vi "Create.vi"(6 "Label Names":string[](array[string]), 7 "Registry Name":string, 8 "error in (no error)":errorcluster) -> (0 "error out":errorcluster, 3 "Process Collector out":refnum<class "Process Collector.lvclass">)   [LabVIEW 2020, in "Collector.lvlib" / "Process Collector.lvclass"]
doc: "Creates a collector for the hosting process. This collector contains CPU and memory information about the process running this code."
uses:
  Process Collector.lvclass
  Process Collector.lvclass/Process Collector.ctl
  metrics/gauge/Gauge.lvclass
  C:/Github-locals/PromVIEW/src/metrics/metric/Metric.lvclass
  <vilib>/regexp/Match Regular Expression.xnode
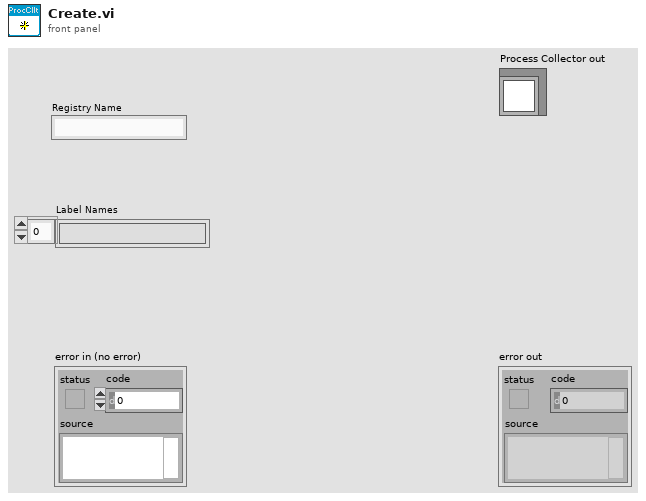
[diagram p1: front panel]
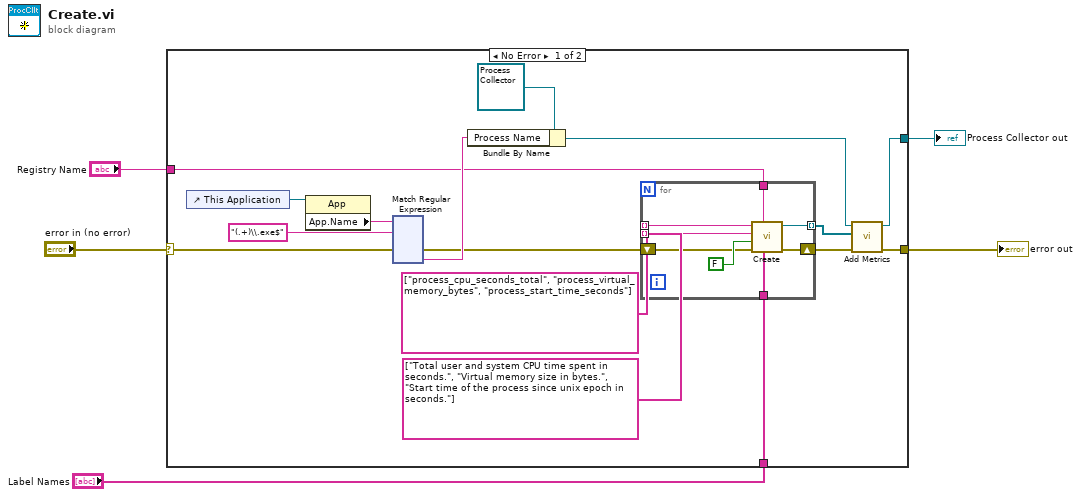
[diagram p0: block diagram]
diagram:
  n1 = case shown="No Error" "error in (no error)" {
    selector: "error in (no error)" -> [w17 w146]
    tunnel: [w8 w146] -> w2
    tunnel: [w9 _] -> w3
    tunnel: "Registry Name" -> [w13 _]
    tunnel: "Label Names" -> [w6 _]
    frame No Error {
      n2 = control-ref of="This Application"() -> (w21:refnum<vi>)
      n3 = property class="App"(reference=w21) -> ("App.Name"=w20:string)  [unwired: 1 in, 2 out]
      n4 = xnode "Match Regular Expression"("input string"=w20, "regular expression"="(.+)\\.exe$", "error in"=w17) -> ("error out"=w12:errorcluster, "submatch 1"=w18:string)  [unwired: 3 in, 4 out]
      n5 = Bundle By Name(cluster=refnum<class "Process Collector.lvclass"> refnum ("Process Collector in"), "Process Name"=w18) -> (w10:refnum<class "Process Collector.lvclass">)
      n6 = for {
        tunnel: string[] ["process_cpu_seconds_total", "process_virtual_memory_bytes", "process_start_time_seconds"] ("Metric Name") -> [w29] mode=indexing
        tunnel: string[] ["Total user and system CPU time spent in seconds.", "Virtual memory size in bytes.", "Start time of the process since unix epoch in seconds."] ("Metric Name") -> [w28] mode=indexing
        tunnel: w13 -> [w27]
        shift-right: [w24] -> w7
        shift-left: w12 -> [w25]
        tunnel: [w23] -> w11 mode=indexing
        tunnel: w6 -> [w22]
        n7 = call "Create.vi"("Label Names"=w22, "Registry Name"=w27, "error in (no error)"=w25, "Auto-register?"=FALSE, "Description"=w28, "Metric Name"=w29) -> ("error out"=w24:errorcluster, "Gauge Ref"=w23:refnum<data-value>)  [unwired: 4 in]
      }
      n8 = call-dynamic "Add Metrics.vi"("error in (no error)"=w7, "Metrics"=w11, "Default Collector in"=w10) -> ("error out"=w8:errorcluster, "Default Collector out"=w9:refnum<class "Process Collector.lvclass">)  [unwired: 7 in]
    }
    frame Error {
    }
  }
  "error out" <- w2
  "Process Collector out" <- w3
